vi "Bat_FPGA.vi"() -> ()   [LabVIEW 2019]
uses:
  <vilib>/rvi/Emulation/niFpgaGetClockAttributes.vi
  <vilib>/rvi/Emulation/niFpgaSctlEmulationGetInTimedLoop.vi
  <vilib>/rvi/Emulation/niFpgaEmulationReportErrorSimple.vi
  <vilib>/rvi/eio/common/nirviEmuTemplateMethod_errors.vi
  <vilib>/rvi/Emulation/niFpgaCriticalErrorInLSC.vi
  <vilib>/eio/EIONode/EIONode.xnode
  <vilib>/rvi/FXPMathLib/FxpMul/XNode/nifxpmath_Multiplier.xnode
  <vilib>/rvi/FXPMathLib/FxpSub/XNode/nifxpmath_Sub.xnode
  <vilib>/rvi/FXPMathLib/sim/FxpSim.dll
panel:
  in  "WaitT(mSec)":u16=100
  in  "T/n*Q":fxp<+,32,1>
  in  "Vmax":fxp<+,12,10>=126.0 format="%#_16g"
  out "number":i16
  out "I_NEED":fxp<+/-,32,16>
  out "Boolean SOC":bool
  in  "1/R0":fxp<+,12,12>
  out "V_bat":fxp<+/-,64,10>
  in  "R0":fxp<+/-,16,1>
  out "ib_rio":fxp<+/-,32,16>
  out "SoC":fxp<+,32,1>
  in  "T*n/Q":fxp<+,32,1>
  in  "SoC(0)":fxp<+,32,1>
  in  "ctrl_SoC":bool
  out "VC2":fxp<+/-,64,7>
  out "VC1":fxp<+/-,64,7>
  in  "s_i":bool
  in  "Ib":fxp<+/-,32,16>
  in  "1-T/(R2C2)":fxp<+,32,0>
  in  "1-T/(R1C1)":fxp<+,32,0>
  in  "T/C2":fxp<+,32,0>
  in  "T/C1":fxp<+,32,0>
  in  "1/(R0+RL)":fxp<+,16,0>
  in  "Voc":fxp<+,32,10>
  out "Time":u32
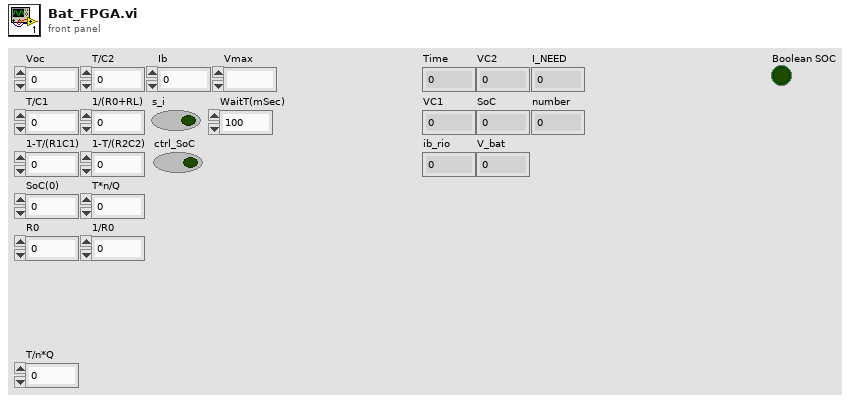
[diagram p1: front panel]
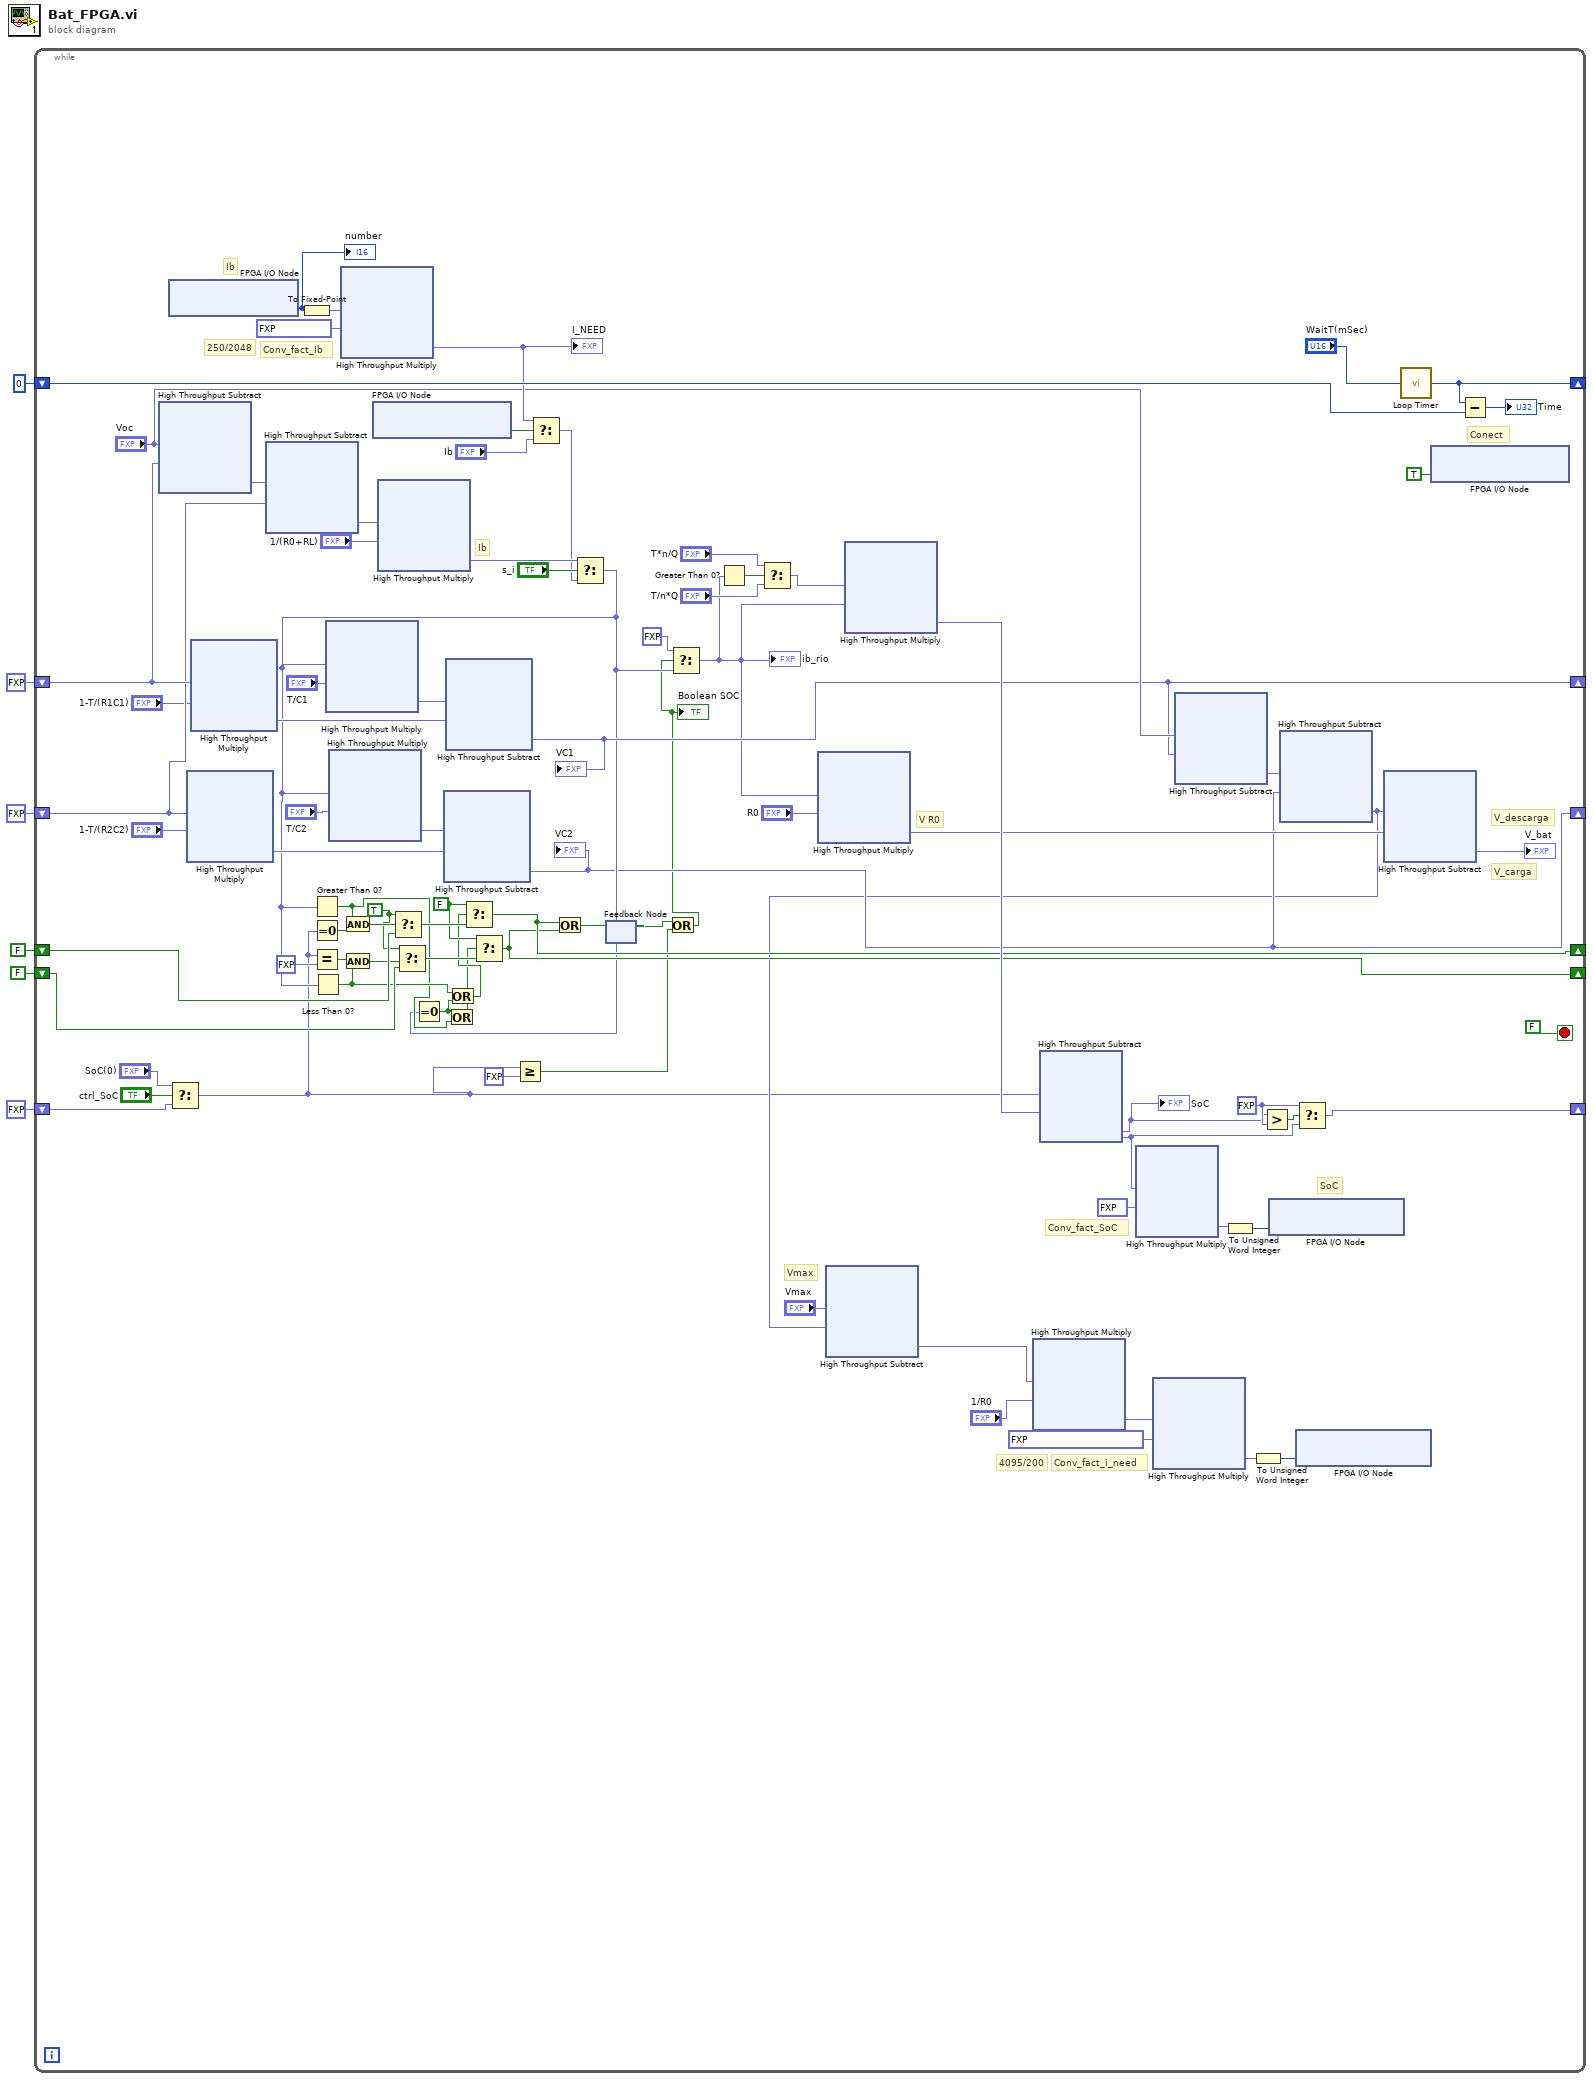
[diagram p0: block diagram]
diagram:
  n1 = while {
    shift-right: [w90] -> _
    shift-left: u32 0 ("Tick Count(mSec)") -> [w89]
    shift-right: [w46] -> _
    shift-left: fxp<+/-,64,7> 0.0 ("x-y") -> [w82]
    shift-right: [w23] -> _
    shift-left: fxp<+/-,64,7> 0.0 ("x-y") -> [w81]
    shift-right: [w52] -> _
    shift-left: fxp<+,32,1> 0.0 ("x+y") -> [w76]
    shift-right: [w32] -> _
    shift-left: FALSE ("t") -> [w39]
    shift-right: [w31] -> _
    shift-left: FALSE ("t") -> [w34]
    stop <- FALSE stop-if-true
    w33 = FALSE ("t")
    w35 = TRUE
    w54 = fxp<+,32,1> 1.0 ("y")
    # "V R0"
    # "4095/200"
    # "Conv_fact_i_need"
    # "Vmax"
    # "V_descarga"
    # "V_carga"
    # "250/2048"
    # "Conv_fact_SoC"
    # "Conv_fact_Ib"
    # "Ib"
    # "SoC"
    # "Conect"
    # "Ib"
    n2 = xnode "High Throughput Subtract"("x"="Voc", "y"=w82) -> ("x-y"=w87:fxp<+/-,64,12>)
    n3 = xnode "FPGA I/O Node"() -> ("ConnectorC/AI0"=w22:i16)  [unwired: 1 in, 1 out]
    "number" <- w22
    n4 = Select(t="SoC(0)", s="ctrl_SoC", f=w76) -> (s? t:f=w11:fxp<+,32,1>)
    n5 = xnode ("High Throughput Multiply")("x"=w81, "y"="1-T/(R2C2)") -> ("x*y"=w84:fxp<+/-,64,7>)
    n6 = xnode ("High Throughput Multiply")("x"=w82, "y"="1-T/(R1C1)") -> ("x*y"=w83:fxp<+/-,64,7>)
    n7 = xnode "High Throughput Subtract"("x"=w87, "y"=w81) -> ("x-y"=w86:fxp<+/-,64,13>)
    n8 = To Fixed-Point(number=w22) -> (fixed-point=w67:fxp<+/-,16,16>)  [unwired: 1 in]
    n9 = Equal To 0?(x=w11) -> (x = 0?=w51:bool)
    n10 = Equal?(x=w11, y=fxp<+,33,1> 1.0) -> (x = y?=w50:bool)
    n11 = xnode ("High Throughput Multiply")("x"=w67, "y"=fxp<+,16,4> 0.1220703125) -> ("x*y"=w63:fxp<+/-,32,16>)
    "I_NEED" <- w63
    n12 = xnode "FPGA I/O Node"() -> ("ConnectorC/DIO7"=w58:bool)  [unwired: 1 in, 1 out]
    n13 = xnode ("High Throughput Multiply")("x"=w86, "y"="1/(R0+RL)") -> ("x*y"=w80:fxp<+/-,32,16>)
    n14 = Greater Or Equal?(x=w11, y=fxp<+,32,1> 1.0) -> (x >= y?=w13:bool)
    n15 = Select(t=w63, s=w58, f="Ib") -> (s? t:f=w7:fxp<+/-,32,16>)
    n16 = Select(t=w80, s="s_i", f=w7) -> (s? t:f=w24:fxp<+/-,32,16>)
    n17 = Greater Than 0?(x=w24) -> (x > 0?=w26:bool)
    n18 = Less Than 0?(x=w24) -> (x < 0?=w28:bool)
    n19 = xnode ("High Throughput Multiply")("x"=w24, "y"="T/C1") -> ("x*y"=w70:fxp<+/-,64,16>)
    n20 = xnode ("High Throughput Multiply")("x"=w24, "y"="T/C2") -> ("x*y"=w69:fxp<+/-,64,16>)
    n21 = And(x=w26, y=w51) -> (x .and. y?=w40:bool)
    n22 = And(x=w50, y=w28) -> (x .and. y?=w37:bool)
    n23 = Select(t=w35, s=w40, f=w39) -> (s? t:f=w38:bool)
    n24 = Select(t=w35, s=w37, f=w34) -> (s? t:f=w36:bool)
    n25 = Equal To 0?(x=w24) -> (x = 0?=w29:bool)
    n26 = xnode "High Throughput Subtract"("x"=w69, "y"=w84) -> ("x-y"=w23:fxp<+/-,64,7>)
    "VC2" <- w23
    n27 = xnode "High Throughput Subtract"("x"=w70, "y"=w83) -> ("x-y"=w46:fxp<+/-,64,7>)
    "VC1" <- w46
    n28 = Or(x=w29, y=w26) -> (x .or. y?=w25:bool)
    n29 = Or(x=w28, y=w29) -> (x .or. y?=w27:bool)
    n30 = Select(t=w33, s=w27, f=w38) -> (s? t:f=w32:bool)
    n31 = Select(t=w33, s=w25, f=w36) -> (s? t:f=w31:bool)
    n32 = Or(x=w32, y=w31) -> (x .or. y?=w30:bool)
    n33 = feedback-in #1(w30) -> ()
    n34 = feedback #1() -> (w12:bool)  [unwired: 1 in]
    n35 = Or(x=w12, y=w13) -> (x .or. y?=w9:bool)
    "Boolean SOC" <- w9
    n36 = Select(t=fxp<+/-,32,16> 0.0 ("f"), s=w9, f=w24) -> (s? t:f=w15:fxp<+/-,32,16>)
    "ib_rio" <- w15
    n37 = Greater Than 0?(x=w15) -> (x > 0?=w18:bool)
    n38 = Select(t="T*n/Q", s=w18, f="T/n*Q") -> (s? t:f=w14:fxp<+,32,1>)
    n39 = xnode ("High Throughput Multiply")("x"=w15, "y"="R0") -> ("x*y"=w57:fxp<+/-,48,17>)
    n40 = xnode ("High Throughput Multiply")("x"=w14, "y"=w15) -> ("x*y"=w75:fxp<+/-,64,17>)
    n41 = xnode "High Throughput Subtract"("x"=w11, "y"=w75) -> ("x-y"=w53:fxp<+,32,1>)
    "SoC" <- w53
    n42 = xnode ("High Throughput Multiply")("x"=w53, "y"=fxp<+,12,12> 4095.0) -> ("x*y"=w64:fxp<+,44,13>)
    n43 = xnode "High Throughput Subtract"("x"="Voc", "y"=w46) -> ("x-y"=w59:fxp<+/-,64,12>)
    n44 = To Unsigned Word Integer(number=w64) -> (unsigned 16bit integer=w61:u16)
    n45 = Greater?(x=w53, y=w54) -> (0:w55:bool)
    n46 = xnode "FPGA I/O Node"("ConnectorA/AO0"=w61) -> ()  [unwired: 1 in, 1 out]
    n47 = xnode "High Throughput Subtract"("x"=w59, "y"=w23) -> ("x-y"=w20:fxp<+/-,64,13>)
    n48 = xnode "High Throughput Subtract"("x"="Vmax", "y"=w20) -> ("x-y"=w19:fxp<+/-,64,14>)
    n49 = xnode ("High Throughput Multiply")("x"=w19, "y"="1/R0") -> ("x*y"=w44:fxp<+/-,64,26>)
    n50 = xnode ("High Throughput Multiply")("x"=w44, "y"=fxp<+,32,12> 20.475000381469727) -> ("x*y"=w42:fxp<+/-,64,38>)
    n51 = To Unsigned Word Integer(number=w42) -> (unsigned 16bit integer=w43:u16)
    n52 = xnode "FPGA I/O Node"("ConnectorA/AO1"=w43) -> ()  [unwired: 1 in, 1 out]
    n53 = Select(t=w54, s=w55, f=w53) -> (s? t:f=w52:fxp<+,32,1>)
    n54 = xnode "High Throughput Subtract"("x"=w20, "y"=w57) -> ("x-y"=→"V_bat":fxp<+/-,64,10>)
    n55 = call "Loop Timer"("Count(mSec)"="WaitT(mSec)") -> ("Tick Count(mSec)"=w90:u32)
    n56 = xnode "FPGA I/O Node"("ConnectorC/DIO6"=TRUE ("ConnectorC/DIO0")) -> ()  [unwired: 1 in, 1 out]
    n57 = Subtract(x=w90, y=w89) -> (x-y=→"Time":u32)
  }
